vi "Untitled 3 (SubVI).vi"(11 "String":path) -> (3 "Path":path)   [LabVIEW 2018]
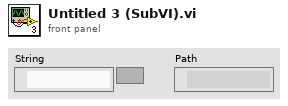
[diagram p1: front panel]
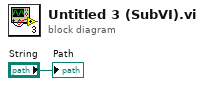
[diagram p0: block diagram]
diagram:
  "Path" <- "String"
